vi "RemoteVI Handle Connection.vi"(0 "connection":u32, 1 "token":string, 5 "html":string, 7 "max clients reached?":bool, 9 "request head":string, 11 "error in":errorcluster) -> (4 "websocket?":bool, 15 "error out":errorcluster)   [LabVIEW 2020, in "RemoteVI.lvlib"]
doc: "Serves ONE HTTP request whose head has been read completely (docs\\protocol.md section 1). The head is read beforehand without blocking by RemoteVI Read Request Head.vi, so this VI never waits for the peer. request head must contain the blank line; it is parsed with IG HTTP Utils Parse From String. The status comes from RemoteVI Route Request.vi (with RemoteVI Cross Origin.vi): GET / and /index.html answer 200 with html and the security headers; /ws answers 426 without a WebSocket upgrade, 403 when an Origin header names another host than Host, 503 when max clients reached? is TRUE, and otherwise the IG WebSocket upgrade response (101) - then websocket? is TRUE and the connection stays open for the caller. Any other path answers 404. Every non-upgrade answer (RemoteVI Send Static Response.vi) closes the connection; a head without the blank line (more than 16 KiB) or one that does not parse is closed without an answer. connection is the TCP connection refnum type-cast to U32 (AIXML has no TCP refnum control type)."
uses:
  RemoteVI.lvlib
  <vilib>/IlluminatedG/IG WebSocket Stream/Stream-Websocket/WebSocketUpgradeResponse/WebSocketUpgradeResponse.lvclass
  <vilib>/IlluminatedG/IG HTTP Utils/HTTP Utils/Request/Request.lvclass
  <vilib>/IlluminatedG/lv-stream/URI/URI.lvclass
  <vilib>/IlluminatedG/IG WebSocket Stream/Stream-Websocket/Stream-Websocket.lvlib
  <vilib>/IlluminatedG/IG HTTP Utils/HTTP Utils/Response/Response.lvclass
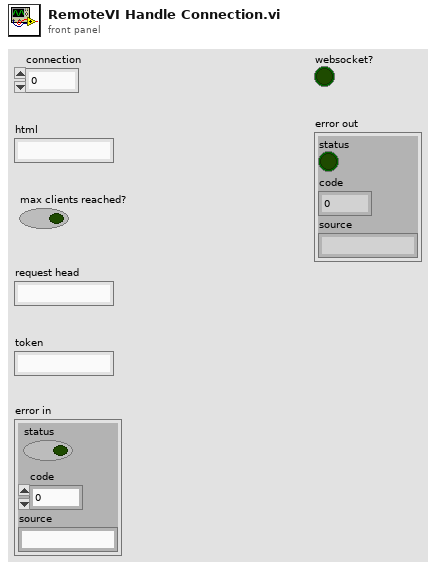
[diagram p1: front panel]
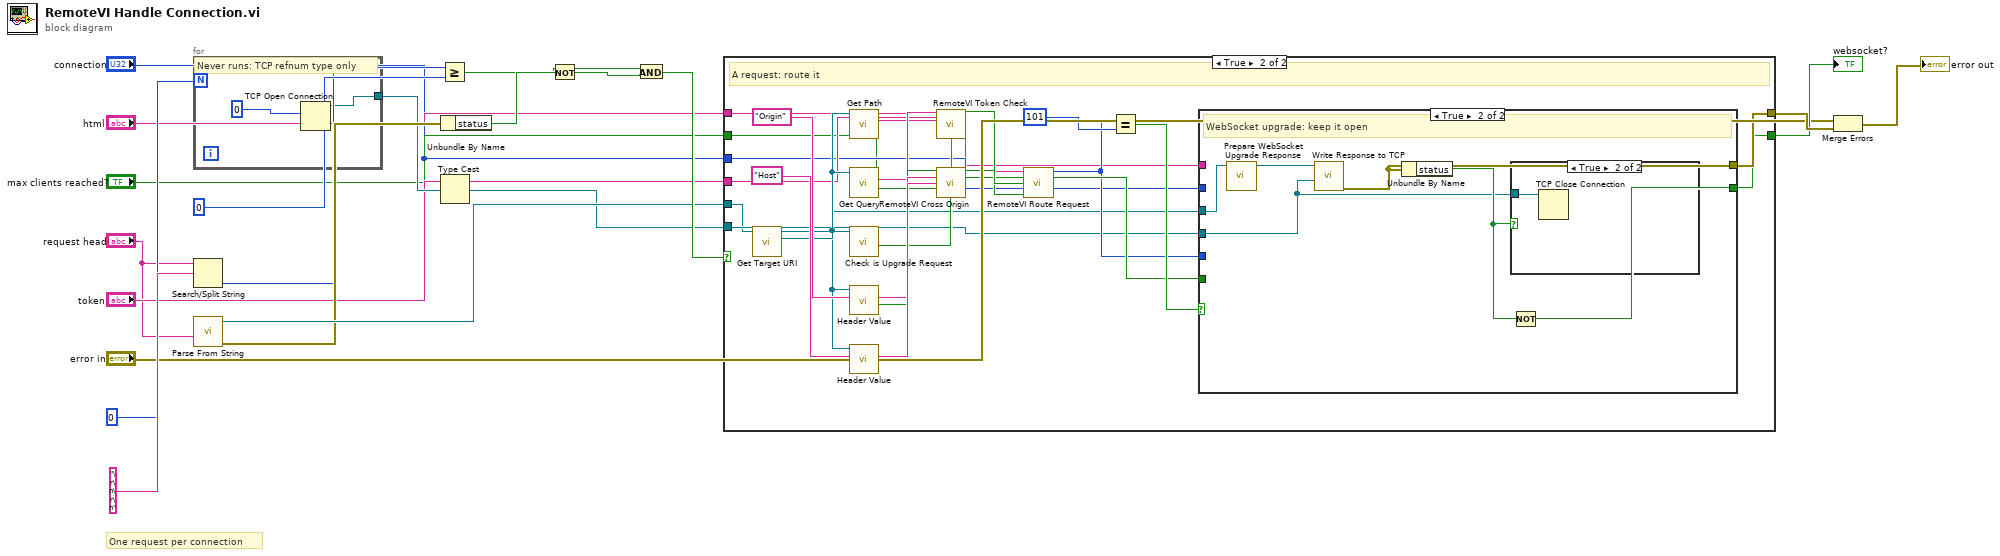
[diagram p0: block diagram]
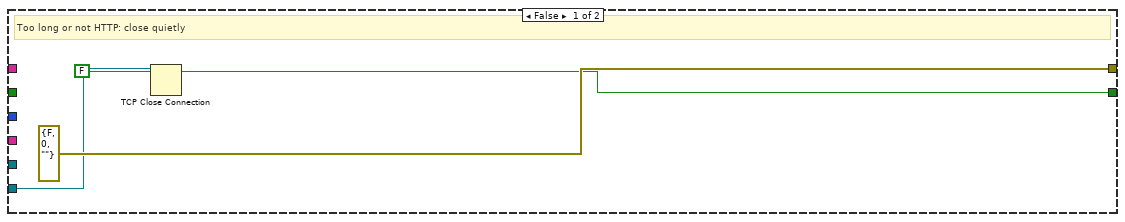
[diagram p2: hidden frame]
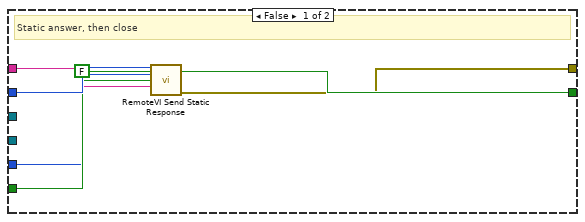
[diagram p3: hidden frame]
diagram:
  # "One request per connection"
  n1 = for {
    N: 0 -> [_]
    tunnel: [w23] -> w8
    # "Never runs: TCP refnum type only"
    n2 = TCP Open Connection(remote port or service name=u16 0) -> (connection ID=w23:refnum<k5>)  [unwired: 4 in, 1 out]
  }
  n3 = Search/Split String(string="request head", search string/char (-)="\r\n\r\n") -> (offset of match=w11:i32)  [unwired: 1 in, 2 out]
  n4 = call <vilib>:"Parse From String.vi"("Request String"="request head") -> ("error out"=w14:errorcluster, "Request out"=w15:refnum<class "Request.lvclass">)  [unwired: 9 in]
  n5 = Greater Or Equal?(x=w11, y=0) -> (x >= y?=w13:bool)
  n6 = Unbundle By Name(w14) -> ("status"=w16:bool)
  n7 = Type Cast(type=w8, x="connection") -> (*(type *) &x=w9:refnum<k5>)
  n8 = Not(x=w16) -> (.not. x?=w17:bool)
  n9 = And(x=w13, y=w17) -> (x .and. y?=w18:bool)
  n10 = case shown="True" w18 {
    tunnel: "html" -> [_ w29]
    tunnel: "max clients reached?" -> [_ w30]
    tunnel: "connection" -> [_ w31]
    tunnel: "token" -> [_ w32]
    tunnel: w15 -> [_ w27]
    tunnel: w9 -> [w24 w28]
    tunnel: [errorcluster {"status"=FALSE, "code"=0, "source"=""} w50] -> w20
    tunnel: [FALSE w49] -> w19
    frame False {
      # "Too long or not HTTP: close quietly"
      n11 = TCP Close Connection(connection ID=w24) -> ()  [unwired: 2 in, 2 out]
    }
    frame True {
      # "A request: route it"
      n12 = call <vilib>:"Get Target URI.vi"("Request in"=w27) -> ("Target URI"=w34:refnum<class "URI.lvclass">, "Request out"=w33:refnum<class "Request.lvclass">)  [unwired: 8 in, 1 out]
      n13 = call <vilib>:"Get Path.vi"("URI in"=w34) -> ("Path"=w35:string)  [unwired: 8 in, 2 out]
      n14 = call <vilib>:"Get Query.vi"("URI in"=w34) -> ("Query"=w36:string)  [unwired: 8 in, 2 out]
      n15 = call <vilib>:"Check is Upgrade Request.vi"("Request in"=w33) -> ("Upgrade Request?"=w38:bool)  [unwired: 7 in, 3 out]
      n16 = call <vilib>:"Header Value.vi"("Header"="Origin", "Request in"=w33) -> ("Exists"=w41:bool, "Value"=w42:string)  [unwired: 6 in, 2 out]
      n17 = call <vilib>:"Header Value.vi"("Header"="Host", "Request in"=w33) -> ("Value"=w43:string)  [unwired: 6 in, 3 out]
      n18 = call "RemoteVI Token Check.vi"("query"=w36, "token"=w32) -> ("ok?"=w37:bool)  [unwired: 13 in]
      n19 = call "RemoteVI Cross Origin.vi"("origin exists?"=w41, "origin"=w42, "host"=w43) -> ("cross origin?"=w44:bool)  [unwired: 12 in]
      n20 = call "RemoteVI Route Request.vi"("path"=w35, "upgrade request?"=w38, "cross origin?"=w44, "max clients reached?"=w30, "token ok?"=w37) -> ("status"=w45:u16, "page?"=w46:bool)  [unwired: 9 in]
      n21 = Equal?(x=w45, y=u16 101) -> (x = y?=w48:bool)
      n22 = case shown="True" w48 {
        tunnel: w29 -> [w53 _]
        tunnel: w31 -> [w54 _]
        tunnel: w33 -> [_ w57]
        tunnel: w28 -> [_ w58]
        tunnel: w45 -> [w51 _]
        tunnel: w46 -> [w52 _]
        tunnel: [w55 w60] -> w50
        tunnel: [FALSE w62] -> w49
        frame False {
          # "Static answer, then close"
          n23 = call "RemoteVI Send Static Response.vi"("connection"=w54, "status"=w51, "page?"=w52, "html"=w53) -> ("error out"=w55:errorcluster)  [unwired: 11 in]
        }
        frame True {
          # "WebSocket upgrade: keep it open"
          n24 = call <vilib>:"Prepare WebSocket Upgrade Response.vi"("Request"=w57) -> ("WebSocket Response"=w59:refnum<class "WebSocketUpgradeResponse.lvclass">)  [unwired: 10 in]
          n25 = call <vilib>:"Write Response to TCP.vi"("TCP Connection"=w58, "Response in"=w59) -> ("error out"=w60:errorcluster)  [unwired: 8 in, 1 out]
          n26 = Unbundle By Name(w60) -> ("status"=w61:bool)
          n27 = case shown="True" w61 {
            tunnel: w58 -> [_ w63]
            frame False {
            }
            frame True {
              n28 = TCP Close Connection(connection ID=w63) -> ()  [unwired: 2 in, 2 out]
            }
          }
          n29 = Not(x=w61) -> (.not. x?=w62:bool)
        }
      }
    }
  }
  "websocket?" <- w19
  n30 = Merge Errors("error in", w20) -> (→"error out":errorcluster)
